vi "user32 GetWindowLongPtrW.vi"(0 "hWnd":u64, 5 "nIndex":i32=-16, 11 "error in":errorcluster) -> (4 "return value":i64, 15 "error out":errorcluster)   [LabVIEW 2020, in "RemoteVI.lvlib"]
doc: "Reads a value of the window hWnd through user32.dll GetWindowLongPtrW (stdcall, called in any thread). nIndex -16 GWL_STYLE returns the window style (WS_POPUP 0x80000000, WS_CAPTION 0x00C00000, WS_VISIBLE 0x10000000); -20 GWL_EXSTYLE the extended style. 0 can mean failure. When error in carries an error the DLL is not called. Generated by scripts\\Build Win32 Wrappers.vi - do not edit by hand, rebuild it."
uses:
  RemoteVI.lvlib
  user32.dll
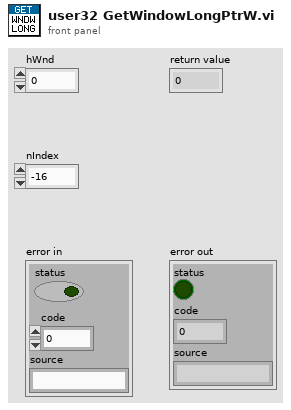
[diagram p1: front panel]
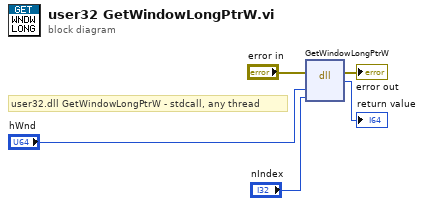
[diagram p0: block diagram]
diagram:
  # "user32.dll GetWindowLongPtrW - stdcall, any thread"
  n1 = dll-call lib="user32.dll" fn="GetWindowLongPtrW"(error in="error in", "hWnd"="hWnd", "nIndex"="nIndex") -> (error out=→"error out":errorcluster, →"return value":i64)  [unwired: 4 in, 1 out]
